vi "Reboot.vi"(8 "error in":errorcluster) -> (0 "error out":errorcluster, 1 "Command Response":string, 2 "Result":string, 3 "RESULT":bool)   [LabVIEW 2021]
uses:
  10054_Control Folder/Support/Relay_no.ctl
  DUT/DUT_Cmd.ctl
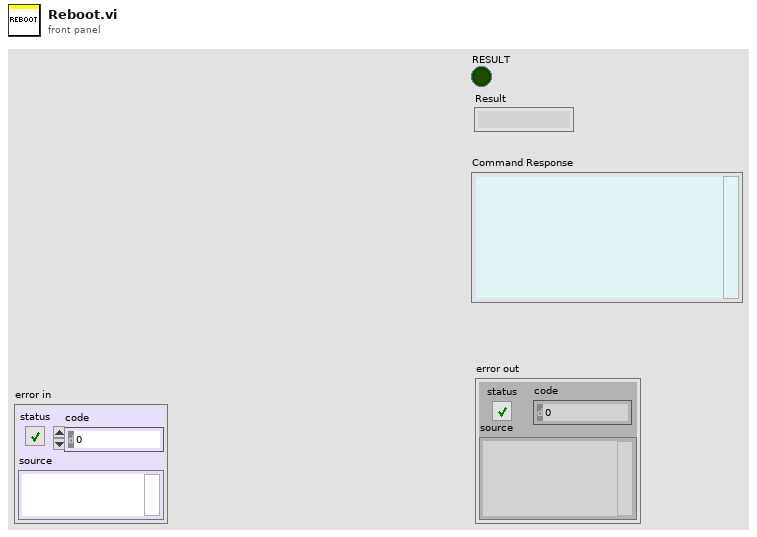
[diagram p1: front panel]
types:
  T1 = typedef "DUT_Cmd.ctl" = enum16{"Unlock serial", "Stop console logs", "Release emergency at start", "Read firmware", "WiFi credentials", "WiFi connected", "WiFi SSID", "Board revision", "ADC_NTC_TEMP", "ADC_TYPE2_RCD_CURRENT", "PCBA serial write", "PCBA serial readback", "Start energy meter", "Energy meter Vac", "Energy meter Iac", "Energy meter PF", "Energy meter energy", "Provision", "Set gateway identity", "CP checklist", "Earth detect", "D+M sense unplugged", "D+M sense plugged", "Output relay weld", "Start diagnostics", "Relay 1 on", "Relay 2 on", "Emergency pressed", "Release emergency", "Emergency released", "Unlock serial for 5 A", "Board current (5 A)", "Unlock serial for 15 A", "Board current (15 A)", "Unlock serial for 0 A", "NFC tag", "Start diagnostics again", "Relay 2 off", "Relay 1 off", "End diagnostics", "Load current (5 A) [No USB station]", "Load current (15 A) [No USB station]", "Load current (0 A) [No USB station]", "NFC tag [No USB station]", "Battery Voltage", "FW Power reset", "Notification LED", "O/P Relay weld Detection", "Earth Detection", "12V ", "5V", "3.3V", "Reboot"}
  T2 = typedef "Relay_no.ctl" = enum16{"Init", "write&Read", "PCB Serial Write & Read", "PCB Write SSD & Password", "Read Wifi state", "Reset", "Close"}
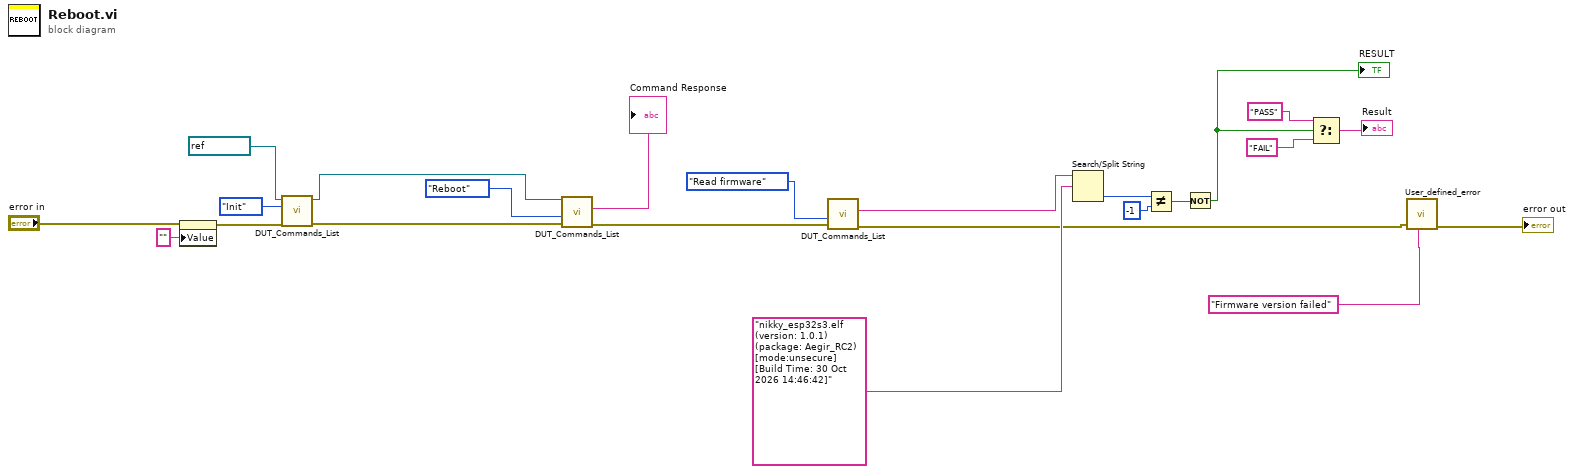
[diagram p0: block diagram]
diagram:
  n1 = property on="Command Response" class="Str"(error in="error in", "Value"="" ("Command Response")) -> (error out=w16:errorcluster)  [unwired: 1 in, 1 out]
  n2 = call "DUT_Commands_List.vi"("error in"=w16, "Operation"=Relay_no."Init", "Resource In"=refnum<visa-resource-name> "COM3") -> ("error out"=w15:errorcluster, "Resource out"=w10:refnum<visa-resource-name>)  [unwired: 6 in, 1 out]
  n3 = call "DUT_Commands_List.vi"("error in"=w15, "DUT Cmd"=DUT_Cmd."Reboot", "Resource In"=w10) -> ("error out"=w4:errorcluster, "Command Response"=→"Command Response":string)  [unwired: 6 in, 1 out]
  n4 = call "DUT_Commands_List.vi"("error in"=w4, "DUT Cmd"=DUT_Cmd."Read firmware") -> ("error out"=w3:errorcluster, "Command Response"=w5:string)  [unwired: 7 in, 1 out]
  n5 = Search/Split String(string=w5, search string/char (-)="nikky_esp32s3.elf (version: 1.0.1) (package: Aegir_RC2) [mode:unsecure] [Build Time: 30 Oct 2026 14:46:42]") -> (offset of match=w7:i32)  [unwired: 1 in, 2 out]
  n6 = Not Equal?(x=w7, y=-1) -> (x != y?=w2:bool)
  n7 = Not(x=w2) -> (.not. x?=w1:bool)
  "RESULT" <- w1
  n8 = Select(t="PASS", s=w1, f="FAIL") -> (s? t:f=→"Result":string)
  n9 = call "User_defined_error.vi"("Error Msg"="Firmware version failed" ("source"), "error in"=w3) -> ("error Out"=→"error out":errorcluster)  [unwired: 9 in]
